vi "Check Consumed.vi"(8 "error in (no error)":errorcluster, 10 "consumed":i32, 11 "size":i32) -> (0 "error out":errorcluster)   [LabVIEW 2021, in "CAN RW CANsub.lvclass"]
uses:
  CAN RW CANsub.lvclass
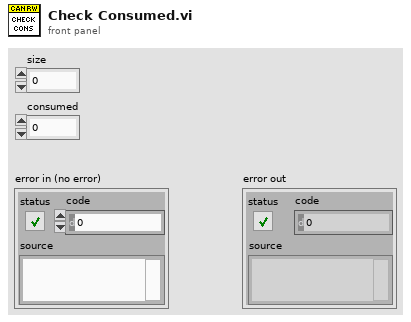
[diagram p1: front panel]
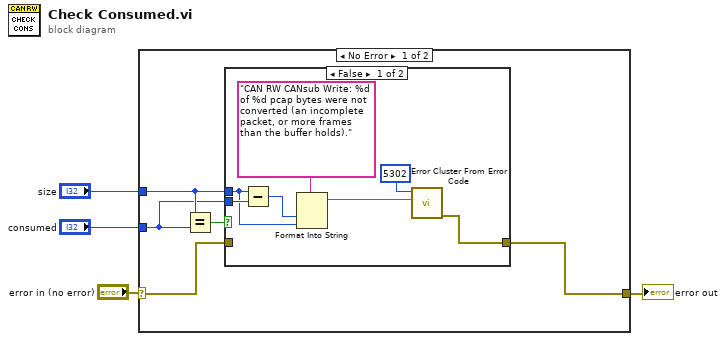
[diagram p0: block diagram]
diagram:
  n1 = case shown="No Error" "error in (no error)" {
    selector: "error in (no error)" -> [w8 w18]
    tunnel: [w7 w18] -> w3
    tunnel: "size" -> [w6 _]
    tunnel: "consumed" -> [w5 _]
    frame No Error {
      n2 = Equal?(x=w6, y=w5) -> (x = y?=w9:bool)
      n3 = case shown="False" w9 {
        tunnel: w8 -> [_ w17]
        tunnel: [w11 w17] -> w7
        tunnel: w6 -> [w10 _]
        tunnel: w5 -> [w16 _]
        frame False {
          n4 = Subtract(x=w10, y=w16) -> (x-y=w14:i32)
          n5 = Format Into String(format string="CAN RW CANsub Write: %d of %d pcap bytes were not converted (an incomplete packet, or more frames than the buffer holds).", w14, w10) -> (resulting string=w13:string)  [unwired: 2 in, 1 out]
          n6 = call <vilib>:"Error Cluster From Error Code.vi"("error message (\"\")"=w13, "error code (0)"=5302) -> ("error out"=w11:errorcluster)  [unwired: 7 in]
        }
        frame True {
        }
      }
    }
    frame Error {
    }
  }
  "error out" <- w3
